vi "Read Boolean Inputs.vi"(8 "error in (no error)":errorcluster, 11 "Modbus in":refnum<class "Modbus.lvclass">) -> (0 "error out":errorcluster, 3 "Modbus out":refnum<class "Modbus.lvclass">)   [LabVIEW 2026, in "Modbus.lvlib" / "Modbus.lvclass"]
uses:
  Modbus.lvclass
  C:/Program Files/National Instruments/LabVIEW 2026/vi.lib/FlexLogger/SDK/PluginSDK.lvlibp/PEFClasses/SDK/Plugin/Plugin.lvclass
  Modbus.lvclass/Modbus.ctl
  <vilib>/FlexLogger/SDK/PluginSDK.lvlibp/PEFClasses/SDK/Plugin/DataHelpers/Write 1D Bool (NChan 1 Sample).vi
  C:/Program Files/National Instruments/LabVIEW 2026/vi.lib/FlexLogger/SDK/PluginSDK.lvlibp/PEFClasses/SDK/Processing Element/Processing Element.lvclass
  D:/Work/FlexLogger/Features/Modbus Plugin/Modbus - Working Copy/Modbus/Modbus.lvclass
  <vilib>/FlexLogger/SDK/PluginSDK.lvlibp/PEFClasses/SDK/Plugin/Plugin.lvclass
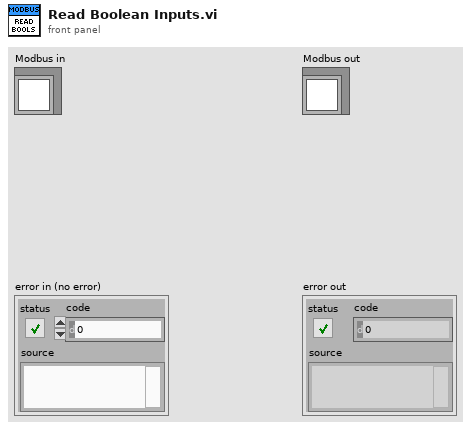
[diagram p1: front panel]
types:
  T1 = typedef "Modbus.lvlib/Modbus.lvclass/Boolean Data.ctl" = cluster{"Channel UID":string, "Valid?":bool, "Table":T2, "Address":i32}
  T2 = typedef "Modbus.lvlib/Modbus.lvclass/Modbus Table.ctl" = enum16{"Discrete Inputs", "Coils", "Input Registers", "Holding Registers"}
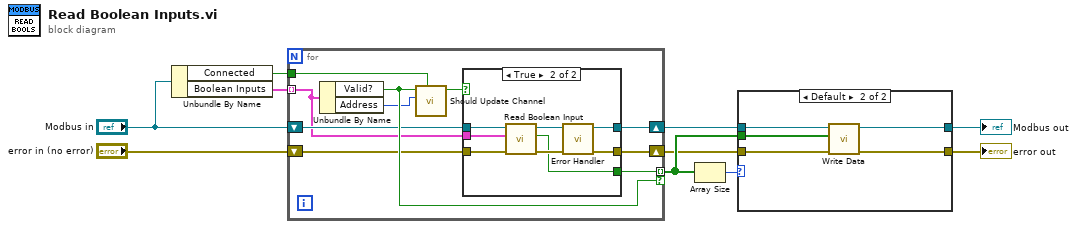
[diagram p0: block diagram]
diagram:
  n1 = Unbundle By Name("Modbus in") -> ("Connected"=w6:bool, "Boolean Inputs"=w3:T1[])
  n2 = for {
    tunnel: w3 -> [w12] mode=indexing
    tunnel: [w20] -> w10 mode=indexing if=w18
    shift-right: [w15] -> w9
    shift-left: "error in (no error)" -> [w17]
    tunnel: w6 -> [w16]
    shift-right: [w13] -> w5
    shift-left: "Modbus in" -> [w14]
    n3 = Unbundle By Name(w12) -> ("Valid?"=w18:bool, "Address"=w11:i32)
    n4 = call "Should Update Channel.vi"("Connected?"=w16, "Address"=w11, "Valid?"=w18) -> ("Update?"=w19:bool)  [unwired: 8 in]
    n5 = case shown="True" w19 {
      tunnel: [w22 w30] -> w15
      tunnel: [_ w23] -> w20
      tunnel: w17 -> [w22 w25]
      tunnel: w14 -> [w21 w28]
      tunnel: [w21 w29] -> w13
      tunnel: w12 -> [_ w24]
      frame False {
      }
      frame True {
        n6 = call "Read Boolean Input.vi"("error in (no error)"=w25, "Boolean Input in"=w24, "Modbus in"=w28) -> ("error out"=w26:errorcluster, "Boolean value"=w23:bool, "Modbus out"=w27:refnum<class "Modbus.lvclass">)  [unwired: 6 in]
        n7 = call "Error Handler.vi"("error in (no error)"=w26, "Modbus in"=w27) -> ("error out"=w30:errorcluster, "Modbus out"=w29:refnum<class "Modbus.lvclass">)  [unwired: 8 in]
      }
    }
  }
  n8 = Array Size(array=w10) -> (size(s)=w4:i32)
  n9 = case shown="Default" w4 {
    tunnel: w5 -> [w32 w37]
    tunnel: w10 -> [_ w36]
    tunnel: w9 -> [w31 w35]
    tunnel: [w32 w34] -> w8
    tunnel: [w31 w33] -> w7
    frame 0 {
    }
    frame Default {
      n10 = call-poly <vilib>:"Write Data.vi"("error in (no error)"=w35, "Data"=w36, "Plugin in"=w37) -> ("error out"=w33:errorcluster, "Plugin out"=w34:refnum<class "Modbus.lvclass">)  [unwired: 7 in]
    }
  }
  "Modbus out" <- w8
  "error out" <- w7
